vi "SeqEditor_StepMLSTaddfromDEFlist.vi"(8 "error in (no error)":errorcluster, 9 "Double-Clicked Row":variant, 11 "NLTest in":refnum<class "NLTest.lvclass">) -> (0 "error out":errorcluster, 3 "NLTest out":refnum<class "NLTest.lvclass">)   [LabVIEW 2017, in "NLTest.lvclass"]
uses:
  NLTest.lvclass
  NLTest.lvclass/NLTest.ctl
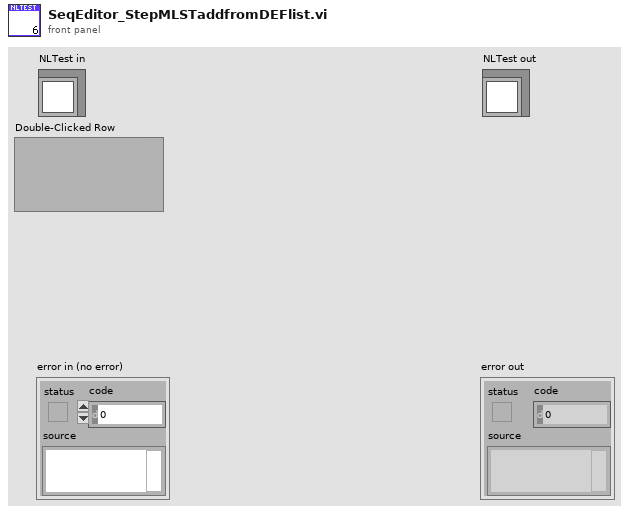
[diagram p1: front panel]
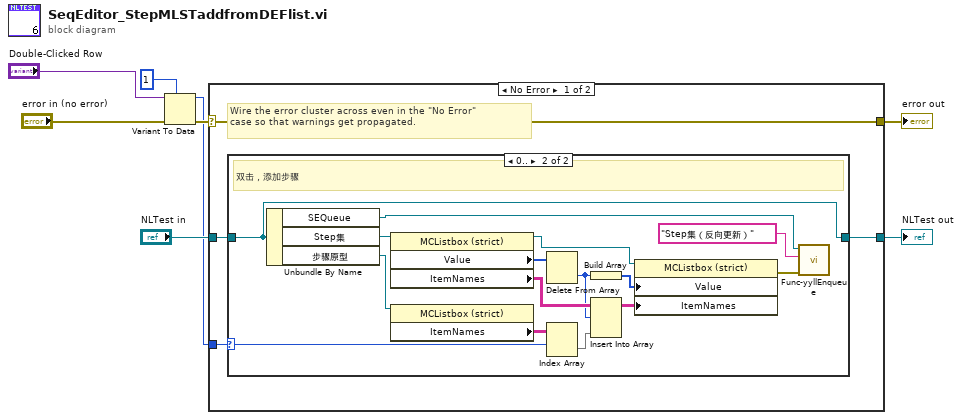
[diagram p0: block diagram]
diagram:
  n1 = Variant To Data(error in="error in (no error)", type=1 ("Get Double-Clicked Row"), Variant="Double-Clicked Row") -> (data=w1:i32, error out=w4:errorcluster)
  n2 = case shown="No Error" w4 {
    selector: w4 -> [w12 w30]
    tunnel: [w12 w30] -> w7
    tunnel: [w9 w29] -> w5
    tunnel: "NLTest in" -> [w10 w29]
    tunnel: w1 -> [w11 _]
    frame No Error {
      # "Wire the error cluster across even in the \"No Error\"\ncase so that warnings get propagated."
      n3 = case shown="0.." w11 {
        selector: w11 -> [_ w25]
        tunnel: w10 -> [w13 w28]
        tunnel: [w13 w28] -> w9
        frame Default {
        }
        frame 0.. {
          # "双击，添加步骤"
          n4 = Unbundle By Name(w28) -> ("SEQueue"=w15:refnum<queue>, "Step集"=w24:refnum<vi>, "步骤原型"=w27:refnum<vi>)
          n5 = property class="MCListbox (strict)"(reference=w24) -> (reference out=w20:refnum<vi>, "Value"=w23:i32[], "ItemNames"=w22:string[][])  [unwired: 1 in, 1 out]
          n6 = property class="MCListbox (strict)"(reference=w27) -> ("ItemNames"=w26:string[][])  [unwired: 1 in, 2 out]
          n7 = Delete From Array(array=w23) -> (deleted portion=w18:i32)  [unwired: 2 in, 1 out]
          n8 = Index Array(array=w26, index (row)=w25) -> (element=w21:string[])  [unwired: 1 in]
          n9 = Build Array(w18) -> (w17:i32[])
          n10 = Insert Into Array(array=w22, index (row)=w18, new element=w21) -> (w19:string[][])  [unwired: 1 in]
          n11 = property class="MCListbox (strict)"(reference=w20, "Value"=w17, "ItemNames"=w19) -> (error out=w14:errorcluster)  [unwired: 1 in, 1 out]
          n12 = call "Func-yyllEnqueue.vi"("error in (no error)"=w14, "cmd"="Step集（反向更新）", "queue in"=w15) -> ()  [unwired: 6 in, 3 out]
        }
      }
    }
    frame Error {
    }
  }
  "error out" <- w7
  "NLTest out" <- w5
